vi "例程53-定义控件粘贴图片.vi"() -> ()   [LabVIEW 2016]
panel:
  in  "停止":bool
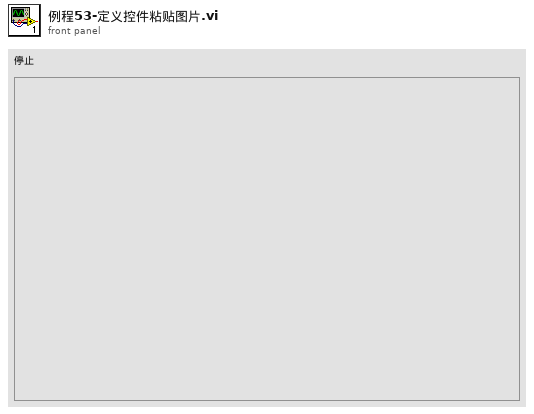
[diagram p1: front panel]
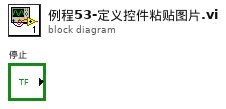
[diagram p0: block diagram]
diagram:
